vi "Sync.vi"(8 "error in (no error)":errorcluster, 10 "file ref":refnum<file>, 11 "rollover trigger in":refnum<class "RolloverTrigger.Age.lvclass">) -> (0 "error out":errorcluster, 3 "rollover trigger out":refnum<class "RolloverTrigger.Age.lvclass">)   [LabVIEW 2018, in "GLog.lvlib" / "RolloverTrigger.Age.lvclass"]
doc: "Synchronizes the rollover trigger with the new file."
uses:
  RolloverTrigger.Age.lvclass
  RolloverTrigger.Age.lvclass/RolloverTrigger.Age.ctl
panel:
  # "Connector Pane"
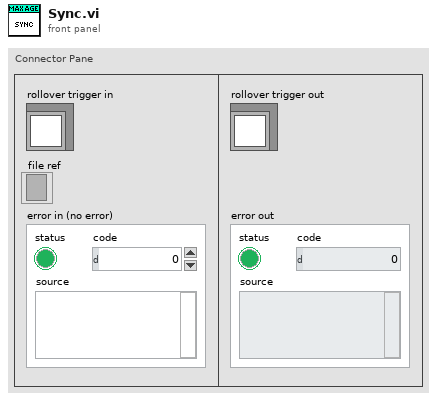
[diagram p1: front panel]
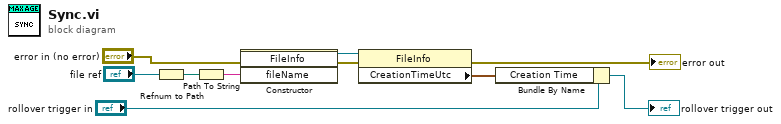
[diagram p0: block diagram]
diagram:
  n1 = Refnum to Path(1:"file ref") -> (0:w8:path)
  n2 = Path To String(path=w8) -> (string=w9:string)
  n3 = constructor class="FileInfo"(error in="error in (no error)", "fileName"=w9) -> (reference out=w10:refnum<k24>, error out=w3:errorcluster)  [unwired: 2 in, 2 out]
  n4 = property class="FileInfo"(reference=w10, error in=w3) -> (error out=→"error out":errorcluster, "CreationTimeUtc"=w4:timestamp)  [unwired: 1 out]
  n5 = Bundle By Name(cluster="rollover trigger in", "Creation Time"=w4) -> (→"rollover trigger out":refnum<class "RolloverTrigger.Age.lvclass">)
